vi "StateMachine_LIDAR.vi"() -> ()   [LabVIEW 2017]
uses:
  <vilib>/myRIO/Instrument Drivers/Onboard IO/DIO/typedefs/DIO Reference.ctl
  <vilib>/myRIO/Common/Instrument Driver Framework/Utilities/typedefs/myRIO Generic Hardware Reference.ctl
  <vilib>/myRIO/Common/Instrument Driver Framework/Utilities/typedefs/Hardware Version Enum.ctl
  <vilib>/myRIO/Common/Instrument Driver Framework/Utilities/typedefs/myRIO v1.0 Reference.ctl
  <vilib>/myRIO/Common/Instrument Driver Framework/Utilities/typedefs/Generic FPGA Reference.ctl
  <vilib>/myRIO/Common/Instrument Driver Framework/myRIO v1.0/DIO/typedefs/DIO Channels List.ctl
  <vilib>/myRIO/Common/Instrument Driver Framework/myRIO v1.0/DIO/typedefs/DIO Channels Enum.ctl
  <vilib>/userdefined/High Color/nirio_resource_hc.ctl
  enum_data_lidar.ctl
  <vilib>/myRIO/Common/Instrument Driver Framework/Utilities/vis/Is FPGA Ref Available.vi
  <vilib>/myRIO/Common/Instrument Driver Framework/myRIO v1.0/DIO/vis/myRIO v1.1 Open DIO.vi
  <vilib>/myRIO/Instrument Drivers/Onboard IO/DIO/vis/Write.vi
  <vilib>/myRIO/Common/Instrument Driver Framework/Utilities/vis/Validate Channels.vi
  <vilib>/myRIO/Common/Instrument Driver Framework/myRIO v1.0/DIO/vis/myRIO v1.0 Reserve DIO.vi
  <vilib>/myRIO/Common/Instrument Driver Framework/myRIO v1.0/Resource Manager/vis/myRIO v1.0 Reserve Channel List.vi
  <vilib>/myRIO/Common/Instrument Driver Framework/myRIO v1.0/DIO/vis/myRIO v1.0 Build MUX Configuration DIO.vi
  <vilib>/myRIO/Common/Instrument Driver Framework/myRIO v1.0/Resource Manager/vis/myRIO v1.0 Reserve Channel.vi
  <vilib>/myRIO/Common/Instrument Driver Framework/myRIO v1.0/Resource Manager/vis/myRIO v1.0 Unreserve Channel.vi
  <vilib>/myRIO/Common/Instrument Driver Framework/myRIO v1.0/Resource Manager/vis/myRIO v1.0 Create Configuration List.vi
  <vilib>/myRIO/Common/Instrument Driver Framework/myRIO v1.0/Resource Manager/vis/myRIO v1.0 Build Mutex Name.vi
  <vilib>/Utility/VariantDataType/GetNumericInfo.vi
  <vilib>/Utility/error.llb/Error Cluster From Error Code.vi
  <vilib>/myRIO/Common/Instrument Driver Framework/myRIO v1.0/myRIO v1.1 Open.vi
  <vilib>/myRIO/Common/Instrument Driver Framework/Utilities/vis/IO Manager.vi
  <vilib>/myRIO/Common/Instrument Driver Framework/Utilities/vis/Configuration Manager.vi
  <vilib>/myRIO/Common/Instrument Driver Framework/myRIO v1.0/Resource Manager/vis/myRIO v1.0 Configure IO.vi
  <vilib>/myRIO/Common/Instrument Driver Framework/myRIO v1.0/myRIO v1.0 Close.vi
  <vilib>/myRIO/Common/Instrument Driver Framework/myRIO v1.0/DIO/vis/myRIO v1.0 Write DIO.vi
  <vilib>/Instr/_visa.llb/VISA Configure Serial Port (Instr).vi
  <vilib>/myRIO/Express VI/Onboard IO/DO/DO Express VI.xnode
  <vilib>/myRIO/Instrument Drivers/Onboard IO/DIO/vis/myRIO DIO Open.xnode
  <vilib>/myRIO/Instrument Drivers/Onboard IO/DIO/DIO.lvlib
panel:
  out "Graphe XY":cluster{"X":dbl, "Y":dbl}[](graph)
  out "Data":cluster{"Angle":dbl, dbl}[](array[cluster])
  in  "Stop":bool
  out "NbPtsMesure":i32
  out "StartScan OK":bool
  out "Firmware":string
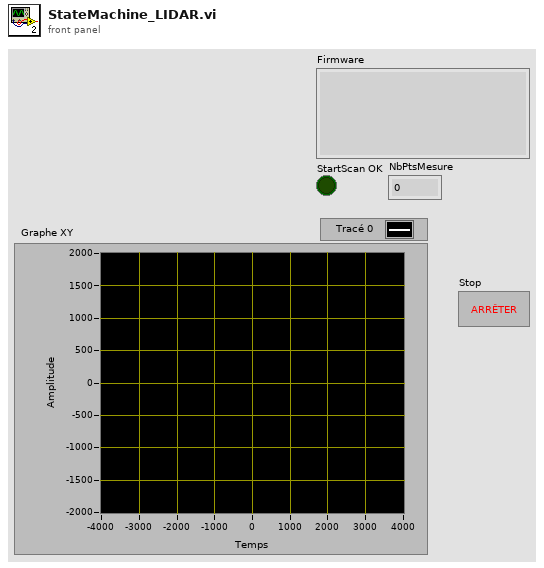
[diagram p1: front panel]
types:
  T1 = typedef "DIO.lvlib/DIO Reference.ctl" = cluster{"myRIO Reference":T2, "DIO Channels List":T6}
  T2 = typedef "myRIO Generic Hardware Reference.ctl" = cluster{"myRIO Model":T3, "myRIO Hardware Reference":T4}
  T3 = typedef "Hardware Version Enum.ctl" = enum16{"Unknown", "myRIO-1900", "myRIO-1950", "roboRIO", "NI ELVIS RIO CM"}
  T4 = typedef "myRIO v1.0 Reference.ctl" = cluster{"Generic FPGA Reference":T5, "Allow multiple opens":bool}
  T5 = typedef "Generic FPGA Reference.ctl" = refnum<k20>
  T6 = typedef "DIO Channels List.ctl" = T7[]
  T7 = typedef "DIO Channels Enum.ctl" = enum16{"Not Connected", "C/DIO0", "C/DIO1", "C/DIO2", "C/DIO3", "C/DIO4", "C/DIO5", "C/DIO6", "C/DIO7", "A/DIO0", "A/DIO1", "A/DIO2", "A/DIO3", "A/DIO4", "A/DIO5", "A/DIO6", "A/DIO7", "A/DIO8", "A/DIO9", "A/DIO10", "A/DIO11", "A/DIO12", "A/DIO13", "A/DIO14", "A/DIO15", "B/DIO0", "B/DIO1", "B/DIO2", "B/DIO3", "B/DIO4", "B/DIO5", "B/DIO6", "B/DIO7", "B/DIO8", "B/DIO9", "B/DIO10", "B/DIO11", "B/DIO12", "B/DIO13", "B/DIO14", "B/DIO15", "LED0", "LED1", "LED2", "LED3", "Button0", "DIO/DIO0", "DIO/DIO1", "DIO/DIO2", "DIO/DIO3", "DIO/DIO4", "DIO/DIO5", "DIO/DIO6", "DIO/DIO7", "DIO/DIO8", "DIO/DIO9", "SPI/CS0", "SPI/CS1", "SPI/CS2", "SPI/CS3", "LED RADIO (Green)", "LED RADIO (Red)", "LED COMM (Green)", "LED COMM (Red)", "LED MODE (Green)", "LED MODE (Red)"}
  T8 = typedef "nirio_resource_hc.ctl" = tag
  T9 = typedef "enum_data_lidar.ctl" = enum16{"Init", "Reset", "Start Scan", "Read Data", "Process Data", "Close"}
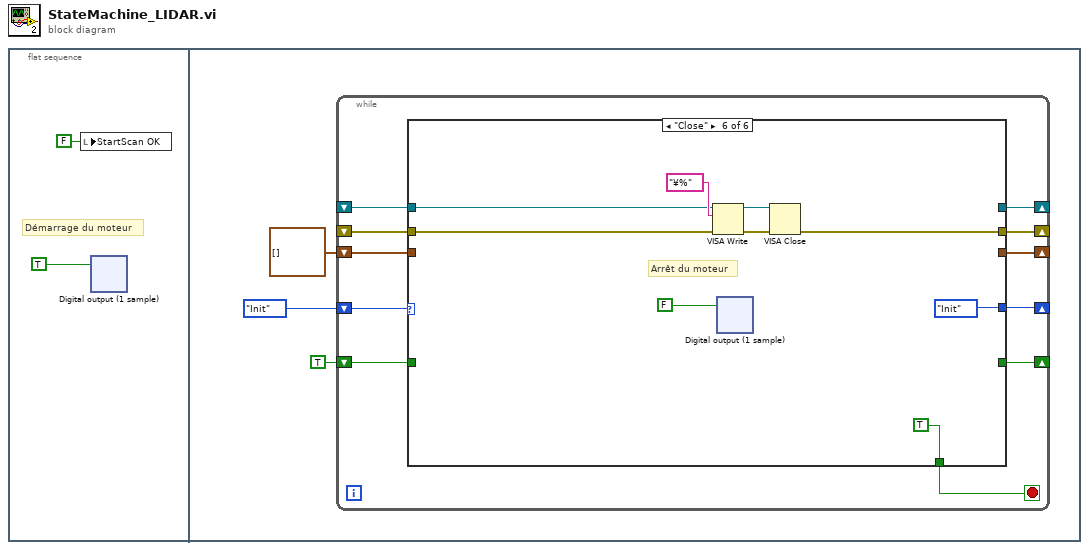
[diagram p0: block diagram]
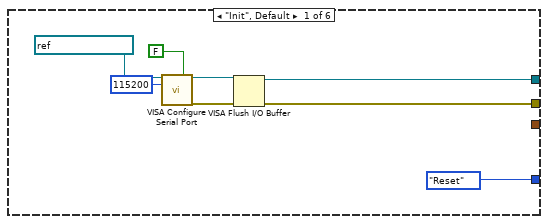
[diagram p2: hidden frame]
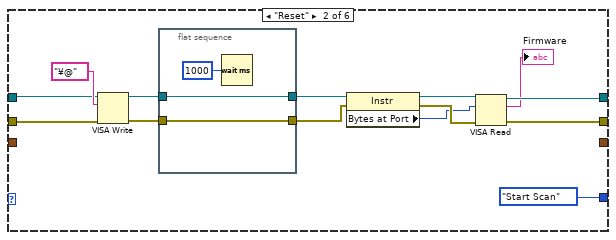
[diagram p3: hidden frame]
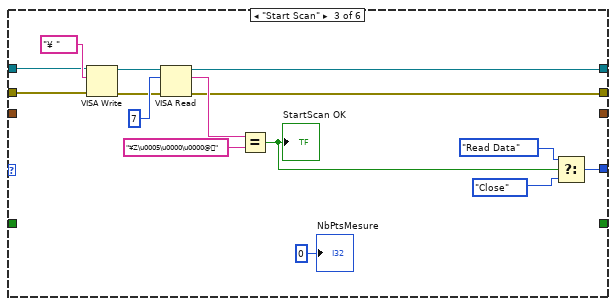
[diagram p4: hidden frame]
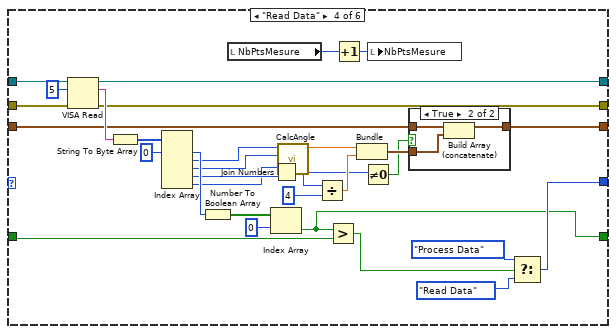
[diagram p5: hidden frame]
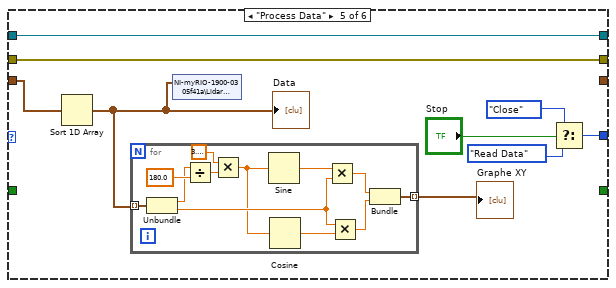
[diagram p7: hidden frame]
diagram:
  n1 = flat-sequence {
    frame #0 {
      # "Démarrage du moteur"
      n2 = local write "StartScan OK"(FALSE ("StartScan OK")) -> ()
      n3 = xnode "Digital output (1 sample)"("B/DIO13 (Pin 26)"=TRUE) -> ()  [unwired: 1 in, 1 out]
    }
    frame #1 {
      n4 = while {
        shift-right: [w46] -> _
        shift-left: enum_data_lidar."Init" ("Etats") -> [w51]
        shift-right: [w50] -> _
        shift-left: _ -> [w48]
        shift-right: [w49] -> _
        shift-left: _ -> [w47]
        shift-right: [w43] -> _
        shift-left: TRUE -> [w44]
        shift-right: [w41] -> _
        shift-left: cluster{"Angle":dbl, dbl}[] [] -> [w42]
        stop <- w45 stop-if-true
        n5 = case shown="\"Close\"" w51 {
          tunnel: [w54 w63 w83 w117 w135 _] -> w50
          tunnel: [w53 w62 w82 w118 w134 w151] -> w49
          tunnel: w48 -> [_ w70 w89 w122 w135 w153]
          tunnel: w47 -> [_ w69 w88 w121 w134 w152]
          tunnel: [enum_data_lidar."Reset" ("Etats") enum_data_lidar."Start Scan" ("Etats") w81 w116 w130 enum_data_lidar."Init" ("Etats")] -> w46
          tunnel: [_ _ _ _ _ TRUE] -> w45
          tunnel: w44 -> [_ _ _ w110 _ _]
          tunnel: [_ _ _ w111 _ _] -> w43
          tunnel: w42 -> [_ _ _ w107 w133 _]
          tunnel: [_ _ _ w106 _ _] -> w41
          frame "Init", Default {
            n6 = call-poly "VISA Configure Serial Port"("VISA resource name"=refnum<visa-resource-name> "ASRL2::INSTR", "Enable Termination\nChar (T)"=FALSE ("Enable Termination\nChar (T)"), "baud rate (9600)"=u32 115200) -> ("VISA resource name out"=w56:refnum<visa-resource-name>, "error out"=w55:errorcluster)  [unwired: 11 in]
            n7 = VISA Flush I/O Buffer(VISA resource name=w56, error in (no error)=w55) -> (VISA resource name out=w54:refnum<visa-resource-name>, error out=w53:errorcluster)  [unwired: 1 in]
          }
          frame "Reset" {
            n8 = VISA Write(VISA resource name=w70, write buffer="¥@" ("Characters to Write"), error in (no error)=w69) -> (VISA resource name out=w73:refnum<visa-resource-name>, error out=w72:errorcluster)  [unwired: 1 out]
            n9 = flat-sequence {
              tunnel: w73 -> [w75]
              tunnel: w72 -> [w74]
              tunnel: [w75] -> w66
              tunnel: [w74] -> w65
              frame #0 {
                n10 = Wait (ms)(milliseconds to wait=u32 1000 ("attente (ms)")) -> ()  [unwired: 1 out]
              }
            }
            n11 = property class="Instr"(reference=w66, error in=w65) -> (reference out=w67:refnum<visa-resource-name>, error out=w68:errorcluster, "Bytes at Port"=w64:u32)
            n12 = VISA Read(VISA resource name=w67, byte count=w64, error in (no error)=w68) -> (VISA resource name out=w63:refnum<visa-resource-name>, read buffer=→"Firmware":string, error out=w62:errorcluster)  [unwired: 1 out]
          }
          frame "Start Scan" {
            n13 = VISA Write(VISA resource name=w89, write buffer="¥ " ("Characters to Write"), error in (no error)=w88) -> (VISA resource name out=w86:refnum<visa-resource-name>, error out=w87:errorcluster)  [unwired: 1 out]
            n14 = VISA Read(VISA resource name=w86, byte count=u32 7 ("nombre d'octets"), error in (no error)=w87) -> (VISA resource name out=w83:refnum<visa-resource-name>, read buffer=w85:string, error out=w82:errorcluster)  [unwired: 1 out]
            n15 = Equal?(x=w85, y="¥Z\u0005\u0000\u0000@") -> (x = y?=w80:bool)
            "StartScan OK" <- w80
            n16 = Select(t=enum_data_lidar."Read Data" ("Etats"), s=w80, f=enum_data_lidar."Close" ("Etats")) -> (s? t:f=w81:T9)
            "NbPtsMesure" <- 0
          }
          frame "Read Data" {
            n17 = VISA Read(VISA resource name=w122, byte count=u32 5 ("nombre d'octets"), error in (no error)=w121) -> (VISA resource name out=w117:refnum<visa-resource-name>, read buffer=w119:string, error out=w118:errorcluster)  [unwired: 1 out]
            n18 = String To Byte Array(string=w119) -> (unsigned byte array=w109:u8[])
            n19 = Index Array(array=w109, index #1=0 ("indice")) -> (element #1=w105:u8, element #2=w104:u8, element #3=w103:u8, element #4=w102:u8, element #5=w101:u8)  [unwired: 4 in]
            n20 = Number To Boolean Array(number=w105) -> (Boolean array=w113:bool[])
            n21 = local read "NbPtsMesure"() -> (w115:i32)
            n22 = Index Array(array=w113, index=0 ("indice")) -> (element=w111:bool)
            n23 = Join Numbers(hi=w101, lo=w102) -> ((hi.lo)=w95:u16)
            n24 = call "CalcAngle.vi"("Octet 2"=w103, "Octet 1"=w104) -> ("Angle"=w100:dbl)  [unwired: 9 in]
            n25 = Divide(x=w95, y=u16 4) -> (x/y=w98:dbl)
            n26 = Greater?(x=w111, y=w110) -> (0:w96:bool)
            n27 = Increment(x=w115) -> (x+1=w114:i32)
            n28 = Bundle("Angle"=w100, w98) -> (w97:cluster{"Angle":dbl, dbl})  [unwired: 1 in]
            n29 = Not Equal To 0?(x=w95) -> (x != 0?=w94:bool)
            n30 = local write "NbPtsMesure"(w114) -> ()
            n31 = case shown="True" w94 {
              tunnel: w107 -> [w123 w126]
              tunnel: [w123 w125] -> w106
              tunnel: w97 -> [_ w124]
              frame False {
              }
              frame True {
                n32 = Build Array (concatenate)(w126, w124) -> (w125:cluster{"Angle":dbl, dbl}[])
              }
            }
            n33 = Select(t=enum_data_lidar."Process Data" ("Etats"), s=w96, f=enum_data_lidar."Read Data" ("Etats")) -> (s? t:f=w116:T9)
          }
          frame "Process Data" {
            n34 = Sort 1D Array(array=w133) -> (sorted array=w127:cluster{"Angle":dbl, dbl}[])
            "Data" <- w127
            n35 = for {
              tunnel: w127 -> [w147] mode=indexing
              tunnel: [w141] -> w132 mode=indexing
              n36 = Unbundle(w147) -> ("Angle"=w137:dbl, w145:dbl)
              n37 = Divide(x=w137, y=180.0) -> (x/y=w139:dbl)
              n38 = Multiply(x=3.141592653589793, y=w139) -> (x*y=w136:dbl)
              n39 = Sine(x=w136) -> (sin(x)=w146:dbl)
              n40 = Cosine(x=w136) -> (cos(x)=w144:dbl)
              n41 = Multiply(x=w146, y=w145) -> (x*y=w143:dbl)
              n42 = Multiply(x=w145, y=w144) -> (x*y=w142:dbl)
              n43 = Bundle(w143, w142) -> (w141:cluster{dbl, dbl})  [unwired: 1 in]
            }
            "Graphe XY" <- w132
            n44 = shared-variable "NI-myRIO-1900-0305f41a\\Lidar Library.lvlib\\Data"(w127) -> ()  [unwired: 1 in, 1 out]
            n45 = Select(t=enum_data_lidar."Close" ("Etats"), s="Stop", f=enum_data_lidar."Read Data" ("Etats")) -> (s? t:f=w130:T9)
          }
          frame "Close" {
            # "Arrêt du moteur"
            n46 = VISA Write(VISA resource name=w153, write buffer="¥%" ("Characters to Write"), error in (no error)=w152) -> (VISA resource name out=w154:refnum<visa-resource-name>, error out=w155:errorcluster)  [unwired: 1 out]
            n47 = xnode "Digital output (1 sample)"("B/DIO13 (Pin 26)"=FALSE) -> ()  [unwired: 1 in, 1 out]
            n48 = VISA Close(VISA resource name=w154, error in (no error)=w155) -> (error out=w151:errorcluster)
          }
        }
      }
    }
  }
